vi "Parse Connect RF Switch Box.vi"(8 "error in (no error)":errorcluster caption="에러 입력(에러 없음)", 10 "JSON string":string, 11 "Instrument Manager 입력":refnum<class "Instrument Manager.lvclass">) -> (0 "error out":errorcluster caption="에러 출력", 1 "Ip Info":cluster{"ip address":string, "port":u16}, 2 "Connect Switch Box Param":T1, 3 "Instrument Manager 출력":refnum<class "Instrument Manager.lvclass">)   [LabVIEW 2023, in "Instrument Manager.lvclass"]
uses:
  Instrument Manager.lvclass
  Param Definition/Connect Switch Box Param.ctl
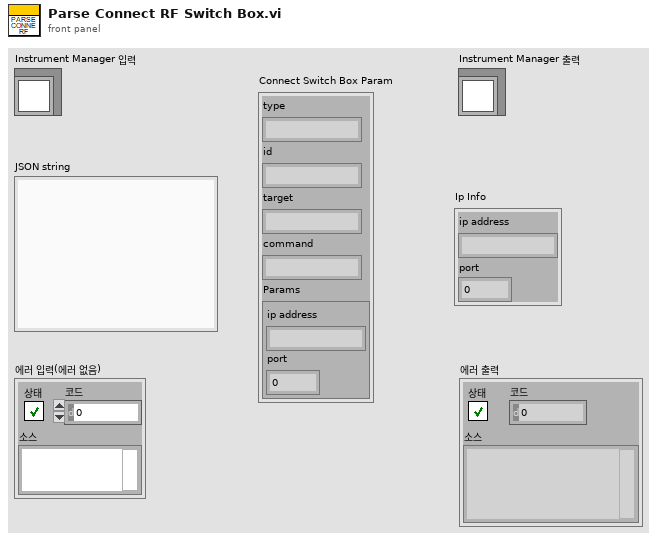
[diagram p1: front panel]
types:
  T1 = typedef "Instrument Manager.lvclass/Connect Switch Box Param.ctl" = cluster{"type":string, "id":string, "target":string, "command":string, "Params":cluster{"ip address":string, "port":i32}}
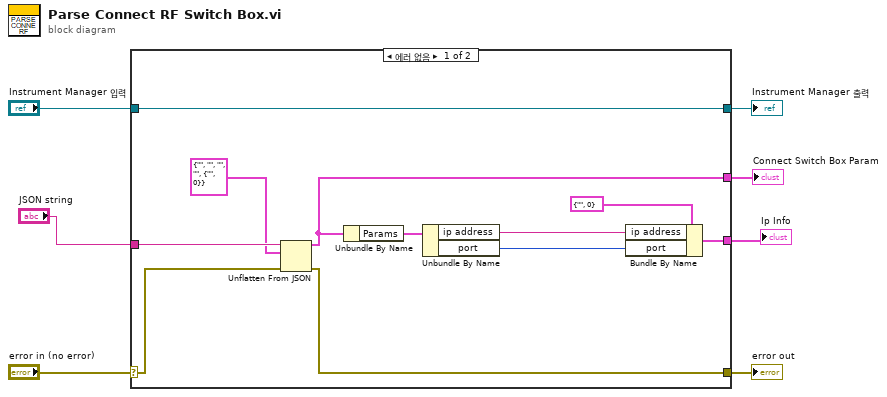
[diagram p0: block diagram]
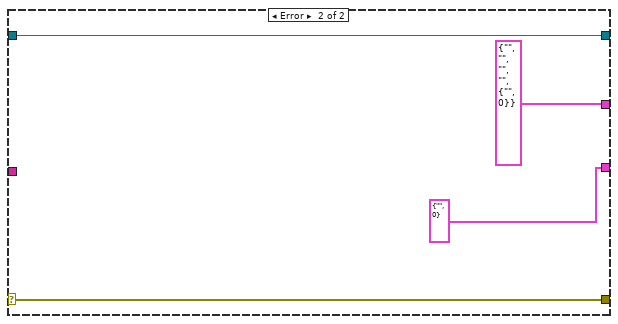
[diagram p2: hidden frame]
diagram:
  n1 = case shown="에러 없음" "error in (no error)" {
    selector: "error in (no error)" -> [w16 w22]
    tunnel: [w15 w22] -> w6
    tunnel: [w18 w21] -> w4
    tunnel: "Instrument Manager 입력" -> [w18 w21]
    tunnel: "JSON string" -> [w17 _]
    tunnel: [w11 T1 {"type"="", "id"="", "target"="", "command"="", "Params"={"ip address"="", "port"=0}} ("Connect Switch Box Param")] -> w2
    tunnel: [w9 cluster{"ip address":string, "port":u16} {"ip address"="", "port"=0} ("Ip Info")] -> w1
    frame No Error {
      n2 = Unflatten From JSON(JSON string=w17, type and defaults=T1 {"type"="", "id"="", "target"="", "command"="", "Params"={"ip address"="", "port"=0}} ("Connect Switch Box Param"), error in (no error)=w16) -> (value=w11:T1, error out=w15:errorcluster)  [unwired: 4 in]
      n3 = Unbundle By Name(w11) -> ("Params"=w12:cluster{"ip address":string, "port":i32})
      n4 = Unbundle By Name(w12) -> ("ip address"=w10:string, "port"=w8:i32)
      n5 = Bundle By Name(cluster=cluster{"ip address":string, "port":u16} {"ip address"="", "port"=0} ("Ip Info"), "ip address"=w10, "port"=w8) -> (w9:cluster{"ip address":string, "port":u16})
    }
    frame Error {
    }
  }
  "error out" <- w6
  "Instrument Manager 출력" <- w4
  "Connect Switch Box Param" <- w2
  "Ip Info" <- w1
